vi "Do Core.vi"(8 "error in (no error)":errorcluster, 9 "Actor in":refnum<class "Actor.lvclass">, 11 "Reply Message":refnum<class "Start Acq Msg.lvclass">) -> (0 "error out":errorcluster, 1 "Actor out":refnum<class "Actor.lvclass">, 2 "Reply":variant)   [LabVIEW 2020, in "DAQ Timed SPIM.lvlib" / "Abstract DAQ Triggered Actor.lvlib" / "Start Acq Msg.lvclass"]
doc: "(<B>Filename</B>: Actor Framework.lvlib:Reply Msg.lvclass:Do Core.vi)\n\nDefines what an actor does when it receives <B>Reply Message</B>. This method also defines the <B>Reply</B> that is returned to the actor that sent <B>Reply Message</B>.\n\nBy default, this method does nothing, and <B>Reply</B> is the ancestor Message class. A child class must override this method to define behavior and specify a child of the Message class to return in the <B>Reply</B> output."
uses:
  Start Acq Msg.lvclass
  <vilib>/ActorFramework/Actor/Actor.lvclass
  Abstract DAQ Triggered Actor/Abstract DAQ Triggered Actor.lvclass
  C:/Program Files/National Instruments/LabVIEW 2020/vi.lib/ActorFramework/Actor/Actor.lvclass
  Start Acq Msg.lvclass/Start Acq Msg.ctl
  fb877dfa-c67d-4f90-8d8a-4d98049191ac.vi
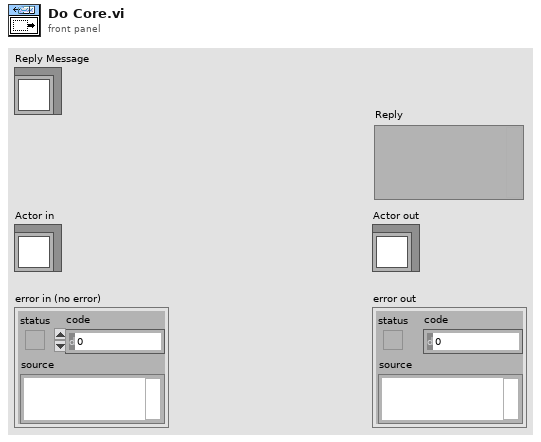
[diagram p1: front panel]
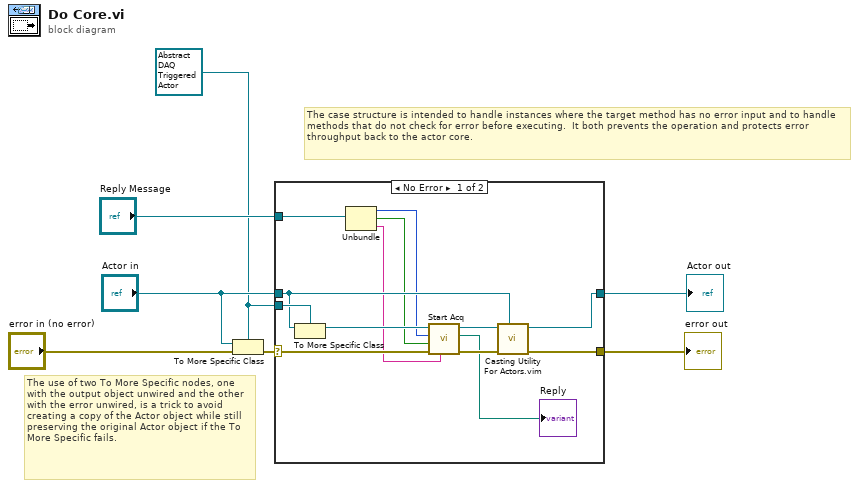
[diagram p0: block diagram]
diagram:
  w2 = refnum<class "Abstract DAQ Triggered Actor.lvclass"> refnum ("DAQ Timed SPIM.lvlib:Abstract DAQ Triggered Actor.lvlib:Abstract DAQ Triggered Actor.lvclass")
  # "The use of two To More Specific nodes, one with the output object unwired and the other with the error unwired, is a trick to avoid creating a copy of the Actor object while still preserving the original Actor object if the To More Specific fails."
  # "The case structure is intended to handle instances where the target method has no error input and to handle methods that do not check for error before executing.  It both prevents the operation and protects error throughput back to the actor core."
  n1 = To More Specific Class(target class=w2, reference="Actor in", error in="error in (no error)") -> (error out=w7:errorcluster)  [unwired: 1 out]
  n2 = case shown="No Error" w7 {
    selector: w7 -> [w16 w22]
    tunnel: [w17 w22] -> w6
    tunnel: [w18 w21] -> w1
    tunnel: "Actor in" -> [w19 w21]
    tunnel: w2 -> [w20 _]
    tunnel: "Reply Message" -> [w13 _]
    frame No Error {
      n3 = To More Specific Class(target class=w20, reference=w19) -> (specific class reference=w12:refnum<class "Abstract DAQ Triggered Actor.lvclass">)  [unwired: 1 in, 1 out]
      n4 = Unbundle(w13) -> (w11:i32, w10:bool, w9:string)
      n5 = call-dynamic "Start Acq.vi"("Filename"=w9, "error in (no error)"=w16, "Write to disk"=w10, "Frame Count"=w11, "Abstract Camera Actor in"=w12) -> ("error out"=w15:errorcluster, "File path"=→"Reply":path, "Abstract Camera Actor out"=w8:refnum<class "Abstract DAQ Triggered Actor.lvclass">)  [unwired: 4 in]
      n6 = call "Casting Utility For Actors.vim"("type"=w19, "error in (no error)"=w15, "Actor in"=w8) -> ("error out"=w17:errorcluster, "Actor out"=w18:refnum<class "Actor.lvclass">)  [unwired: 7 in]
    }
    frame Error {
      # "If type check fails, pass the original object out again."
    }
  }
  "error out" <- w6
  "Actor out" <- w1
